vi "PicoScope4000aGetTimebase2.vi"(4 "Number of Samples":u32, 6 "Memory Segment":u32, 7 "Acquisition Settings":T1 {"postTriggerSamples" format="%_6p"; "preTriggerSamples" format="%_6p"}, 8 "error in (no error)":errorcluster, 11 "handle in":i16) -> (0 "error out":errorcluster, 3 "handle out":i16, 5 "Properties Panel":T2 {"Max Total Capture Time Available (sec)" format="%.3p"; "Sample Frequency" format="%.6p"; "Sample Rate" format="%.3p"; "Max Samples Available" format="%_6p"; "Total Capture Time (sec)" format="%.3p"})   [LabVIEW 2009]
doc: "Calls Gettimebase function"
uses:
  Program Files/Pico Technology/SDK/lib/ps4000a.dll
  shared/Acquisition Settings.ctl
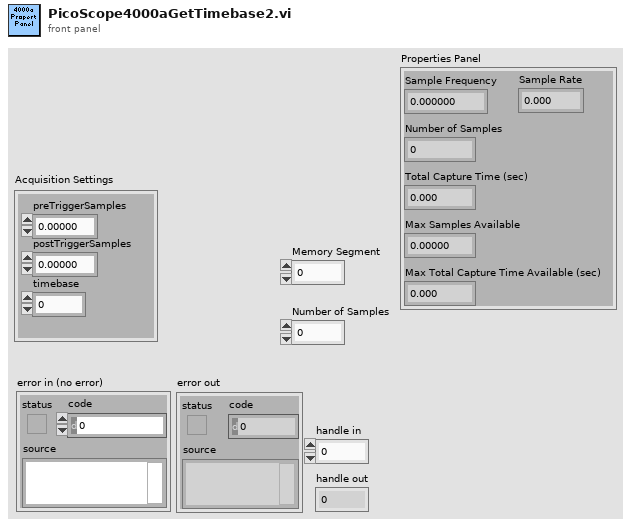
[diagram p1: front panel]
types:
  T1 = typedef "Acquisition Settings.ctl" = cluster{"preTriggerSamples":u64, "postTriggerSamples":u64, "timebase":u32}
  T2 = cluster{"Sample Frequency":dbl, "Sample Rate":dbl, "Max Samples Available":u64, "Number of Samples":u64, "Total Capture Time (sec) ":dbl, "Max Total Capture Time Available (sec)":dbl}
  T3 = cluster{sgl, sgl, "maxSamples":i32, "Number of Samples":u32, sgl, sgl}
  T4 = cluster{"status":bool, "code":u32, "source":string}
  T5 = cluster{dbl, dbl, "maxSamples":i32, "Number of Samples":u32, dbl, dbl}
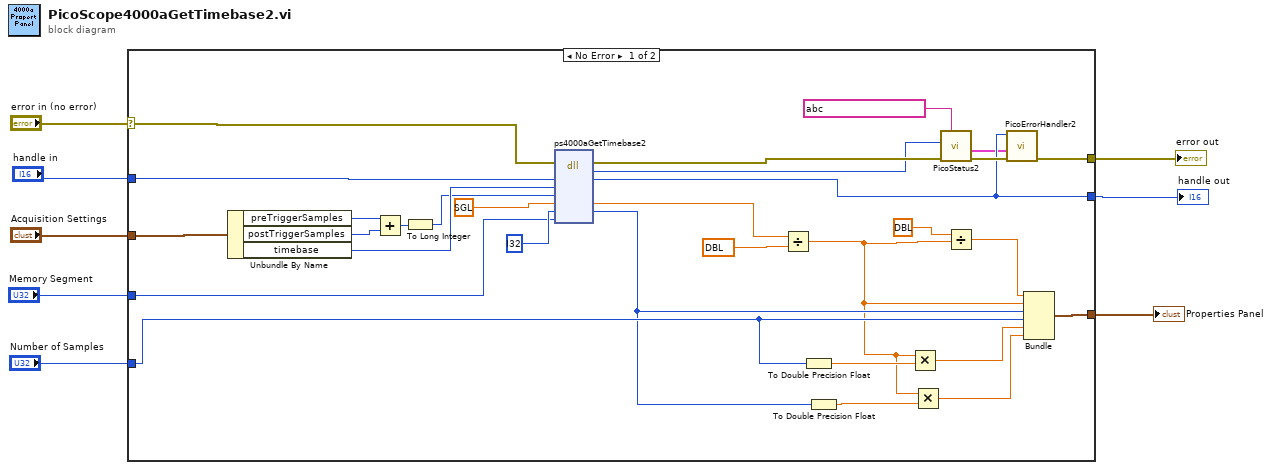
[diagram p0: block diagram]
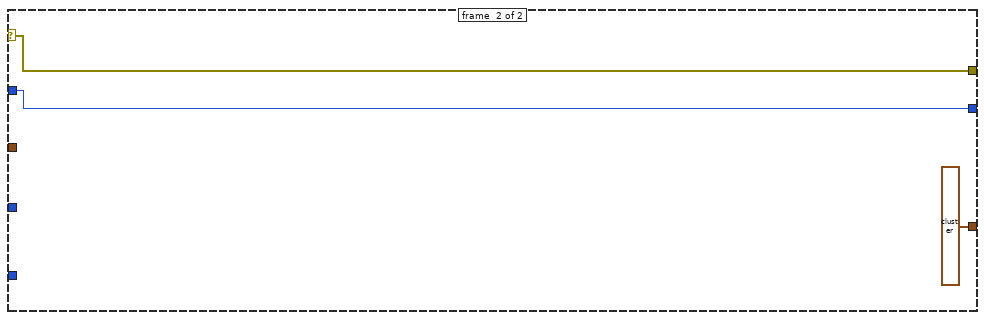
[diagram p2: hidden frame]
diagram:
  n1 = case shown="No Error" "error in (no error)" {
    selector: "error in (no error)" -> [w16 w41]
    tunnel: [w14 w41] -> w8
    tunnel: [w13 w40] -> w7
    tunnel: "Memory Segment" -> [w28 _]
    tunnel: "Number of Samples" -> [w24 _]
    tunnel: "handle in" -> [w27 w40]
    tunnel: [w20 T3 ?] -> w2
    tunnel: "Acquisition Settings" -> [w10 _]
    frame #0 {
      n2 = Unbundle By Name(w10) -> ("preTriggerSamples"=w33:u64, "postTriggerSamples"=w34:u64, "timebase"=w35:u32)
      n3 = Add(x=w33, y=w34) -> (x+y=w12:u64)
      n4 = To Long Integer(number=w12) -> (32bit integer=w11:i32)
      n5 = dll-call lib="/Program Files/Pico Technology/SDK/lib/ps4000a.dll" fn="ps4000aGetTimebase2"(error in=w16, "handle"=w27, "timebase"=w35, "noSamples"=w11, "timeIntervalNanoseconds"=sgl ?, "maxSamples"=i32 ?, "segmentIndex"=w28) -> (error out=w36:errorcluster, "PICO_STATUS"=w29:u32, "handle"=w13:i16, "timeIntervalNanoseconds"=w37:sgl, "maxSamples"=w22:i32)  [unwired: 5 in, 1 out]
      n6 = Divide(x=w37, y=dbl ?) -> (x/y=w19:dbl)
      n7 = To Double Precision Float(number=w24) -> (double precision float=w26:dbl)
      n8 = To Double Precision Float(number=w22) -> (double precision float=w23:dbl)
      n9 = Multiply(x=w19, y=w26) -> (x*y=w25:dbl)
      n10 = Multiply(x=w19, y=w23) -> (x*y=w21:dbl)
      n11 = call "PicoStatus2.vi"("PICO source"=string ? ("source"), "Error in"=w36, "PICO STATUS"=w29) -> ("error out"=w15:errorcluster, "PICO_STATUS out"=w9:T4)  [unwired: 5 in]
      n12 = Divide(x=dbl ?, y=w19) -> (x/y=w17:dbl)
      n13 = call "PicoErrorHandler2.vi"("error in (no error)"=w15, "PICO_STATUS in"=w9, "handle In"=w13) -> ("error out"=w14:errorcluster)  [unwired: 8 in]
      n14 = Bundle(w17, w19, "maxSamples"=w22, "Number of Samples"=w24, w25, w21) -> (w20:T5)  [unwired: 1 in]
    }
    frame #1 {
    }
  }
  "error out" <- w8
  "handle out" <- w7
  "Properties Panel" <- w2
